vi "test Get-Set-Get Label Properties.vi"(8 "error in":errorcluster, 11 "TestCase in":refnum<class "Scripting.lvclass">) -> (0 "error out":errorcluster, 3 "TestCase out":refnum<class "Scripting.lvclass">)   [LabVIEW 2020, in "Scripting.lvclass"]
uses:
  Scripting.lvclass
  Shared/Label Properties.ctl
  Shared/Label.ctl
  Shared/Direction.ctl
  Shared/SDI.ctl
  Shared/Transfer Type.ctl
  Scripting.lvclass/Scripting.ctl
  <vilib>/addons/_JKI Toolkits/VI Tester/TestCase.llb/TestCase.lvclass
  Scripting/AIM/AIM ARINC 429 Scripting.lvlib
  Shared/Transfer Speed.ctl
  C:/Program Files (x86)/National Instruments/LabVIEW 2020/vi.lib/addons/_JKI Toolkits/VI Tester/TestCase.llb/TestCase.lvclass
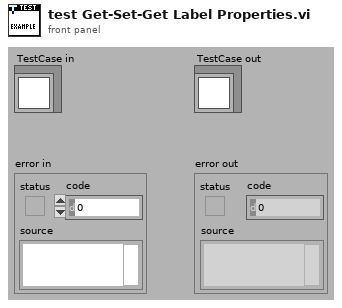
[diagram p1: front panel]
types:
  T1 = typedef "Transfer Type.ctl" = enum16{"Scheduled", "Acyclic", "Block", "Strobe"}
  T2 = typedef "Direction.ctl" = enum16{"Rx", "Tx"}
  T3 = typedef "Transfer Speed.ctl" = enum16{"LO (12.5 kb/s)", "HI (100 kb/s)"}
  T4 = typedef "SDI.ctl" = i32
  T5 = typedef "Label Properties.ctl" = cluster{"label (Dec)":T6, "SDI value":u8, "SDI enabled":bool}
  T6 = typedef "Label.ctl" = u8
  T7 = typedef "Custom Device API.lvlib/Custom Device Item Ref.ctl" = u64
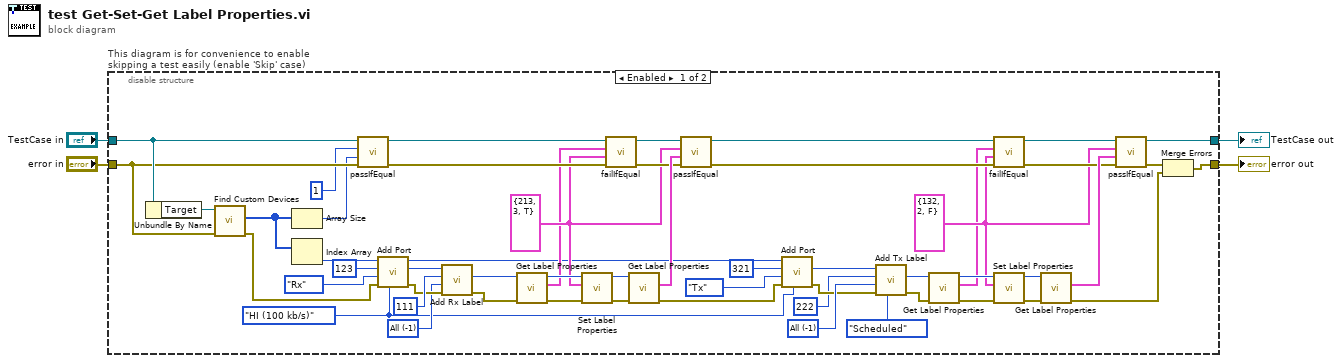
[diagram p0: block diagram]
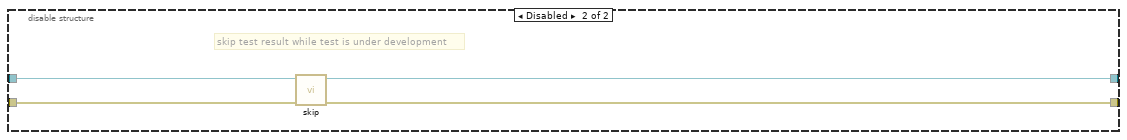
[diagram p2: hidden frame]
diagram:
  n1 = disable-structure "This diagram is for convenience to enable skipping a test easily (enable 'Skip' case)" shown="Enabled" {
    disable-tunnel: "TestCase in" -> [w57 w62]
    disable-tunnel: [w51 w60] -> w1
    disable-tunnel: [w53 w61] -> w3
    disable-tunnel: "error in" -> [w56 w59]
    frame Enabled {
      w5 = Transfer_Speed."HI (100 kb/s)" ("speed")
      w16 = T4 -1 items=["All"=-1, "0 (b00)"=0, "1 (b01)"=1, "2 (b10)"=2, "3 (b11)"=3] ("SDI value")
      w19 = T4 -1 items=["All"=-1, "0 (b00)"=0, "1 (b01)"=1, "2 (b10)"=2, "3 (b11)"=3] ("SDI value")
      w29 = T5 {"label (Dec)"=132, "SDI value"=2, "SDI enabled"=FALSE} ("label properties")
      w35 = T5 {"label (Dec)"=213, "SDI value"=3, "SDI enabled"=TRUE} ("label properties")
      n2 = Unbundle By Name(w57) -> ("Target"=w58:refnum<k24>)
      n3 = call "Find Custom Devices.vi"("error in"=w56, "target in"=w58) -> ("error out"=w25:errorcluster, "AIM ARINC 429 custom devices"=w27:u64[])  [unwired: 7 in, 1 out]
      n4 = Array Size(array=w27) -> (size(s)=w54:i32)
      n5 = Index Array(array=w27) -> (element=w26:u64)  [unwired: 1 in]
      n6 = call-dynamic "passIfEqual.vi"("error in (no error)"=w56, "y"=w54, "x"=1 ("size(s)"), "TestCase in"=w57) -> ("error out"=w38:errorcluster, "TestCase out"=w39:refnum<class "Scripting.lvclass">)  [unwired: 6 in]
      n7 = call "Add Port.vi"("speed"=w5, "error in"=w25, "direction"=Direction."Rx", "port number"=u16 123, "AIM ARINC 429 custom device in"=w26) -> ("error out"=w20:errorcluster, "port"=w22:T7, "AIM ARINC 429 custom device out"=w10:T7)  [unwired: 4 in]
      n8 = call "Add Rx Label.vi"("error in"=w20, "SDI value"=w19, "label value"=u32 111, "port in"=w22) -> ("error out"=w18:errorcluster, "label"=w17:T7)  [unwired: 5 in, 1 out]
      n9 = call "Get Label Properties.vi"("error in"=w18, "label ref in"=w17) -> ("error out"=w49:errorcluster, "label properties"=w34:T5, "label ref out"=w50:T7)  [unwired: 6 in, 1 out]
      n10 = call "Set Label Properties.vi"("error in"=w49, "label properties"=w35, "label ref"=w50) -> ("error out"=w47:errorcluster, "label ref out"=w48:T7)  [unwired: 7 in]
      n11 = call-dynamic "failIfEqual.vi"("error in (no error)"=w38, "y"=w35, "x"=w34, "TestCase in"=w39) -> ("error out"=w36:errorcluster, "TestCase out"=w37:refnum<class "Scripting.lvclass">)  [unwired: 6 in]
      n12 = call "Get Label Properties.vi"("error in"=w47, "label ref in"=w48) -> ("error out"=w9:errorcluster, "label properties"=w46:T5)  [unwired: 6 in, 2 out]
      n13 = call-dynamic "passIfEqual.vi"("error in (no error)"=w36, "y"=w46, "x"=w35, "TestCase in"=w37) -> ("error out"=w32:errorcluster, "TestCase out"=w33:refnum<class "Scripting.lvclass">)  [unwired: 6 in]
      n14 = call "Add Port.vi"("speed"=w5, "error in"=w9, "direction"=Direction."Tx", "port number"=u16 321, "AIM ARINC 429 custom device in"=w10) -> ("error out"=w15:errorcluster, "port"=w13:T7)  [unwired: 4 in, 1 out]
      n15 = call "Add Tx Label.vi"("transfer type"=Transfer_Type."Scheduled", "error in"=w15, "SDI value"=w16, "label value"=u32 222, "port in"=w13) -> ("error out"=w8:errorcluster, "label"=w7:T7)  [unwired: 4 in, 1 out]
      n16 = call "Get Label Properties.vi"("error in"=w8, "label ref in"=w7) -> ("error out"=w43:errorcluster, "label properties"=w28:T5, "label ref out"=w42:T7)  [unwired: 6 in, 1 out]
      n17 = call-dynamic "failIfEqual.vi"("error in (no error)"=w32, "y"=w29, "x"=w28, "TestCase in"=w33) -> ("error out"=w30:errorcluster, "TestCase out"=w31:refnum<class "Scripting.lvclass">)  [unwired: 6 in]
      n18 = call "Set Label Properties.vi"("error in"=w43, "label properties"=w29, "label ref"=w42) -> ("error out"=w45:errorcluster, "label ref out"=w44:T7)  [unwired: 7 in]
      n19 = call "Get Label Properties.vi"("error in"=w45, "label ref in"=w44) -> ("error out"=w41:errorcluster, "label properties"=w40:T5)  [unwired: 6 in, 2 out]
      n20 = call-dynamic "passIfEqual.vi"("error in (no error)"=w30, "y"=w40, "x"=w29, "TestCase in"=w31) -> ("error out"=w52:errorcluster, "TestCase out"=w51:refnum<class "Scripting.lvclass">)  [unwired: 6 in]
      n21 = Merge Errors(w52, w41) -> (w53:errorcluster)
    }
    frame Disabled {
      # "skip test result while test is under development"
      n22 = call <vilib>:"skip.vi"("error in (no error)"=w59, "TestCase in"=w62) -> ("error out"=w61:errorcluster, "TestCase out"=w60:refnum<class "Scripting.lvclass">)  [unwired: 8 in]
    }
  }
  "error out" <- w3
  "TestCase out" <- w1
